vi "drawCircle.vi"(0 "reference":refnum<class "Graphics.lvclass">, 1 "rectangle":T1 {"height" format="%.2f"; "width" format="%.2f"; "y" format="%.2f"; "x" format="%.2f"}, 2 "lineWidth(1)":dbl=1.0 format="%.2f", 3 "color(if not used=default color)":u32=33554432 format="%.0x", 4 "fill?(F)":bool, 5 "error in (no error)":errorcluster) -> (14 "reference out":refnum<class "Graphics.lvclass">, 19 "error out":errorcluster)   [LabVIEW 2020, in "Graphics.lvclass"]
uses:
  <resource>/Framework/Providers/Open_GDS/UML/Graphics_class/Graphics.lvclass
  <resource>/Framework/Providers/Open_GDS/UML/General/Rectangle/Rectangle Rectangle2D.ctl
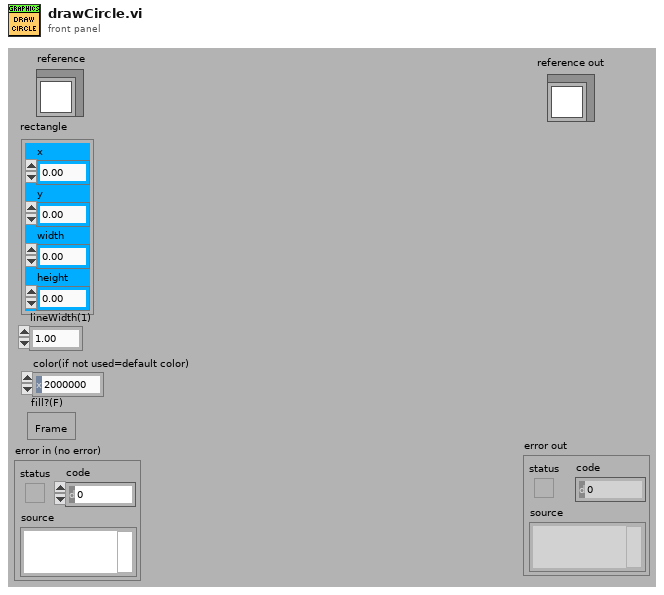
[diagram p1: front panel]
types:
  T1 = typedef "Rectangle Rectangle2D.ctl" = cluster{"x":dbl, "y":dbl, "width":dbl, "height":dbl}
  T2 = typedef "Graphics.lvclass/ObjectAttributes.ctl" = cluster{"drawColor":u32, "backgroundColor":u32, "font":T3, "fontType":T4, "picture":picture, "stroke":T5, "scaleX":dbl, "scaleY":dbl, "screenRef":refnum<vi>, "offsetX":dbl, "offsetY":dbl}
  T3 = typedef "Graphics.lvclass/FontType.ctl" = cluster{"Font Name:":string, "Size":i16, "Strikeout?":bool, "Italic?":bool, "Underline?":bool, "Outline?":bool, "Shadow?":bool, "Bold?":bool}
  T4 = typedef "Graphics.lvclass/LvFontType.ctl" = enum16{"User-specified Font", "Application Font", "System Font", "Dialog Font"}
  T5 = typedef "Graphics.lvclass/StrokeType.ctl" = enum16{"USE_DEFAULT", "SOLID", "DOTTED"}
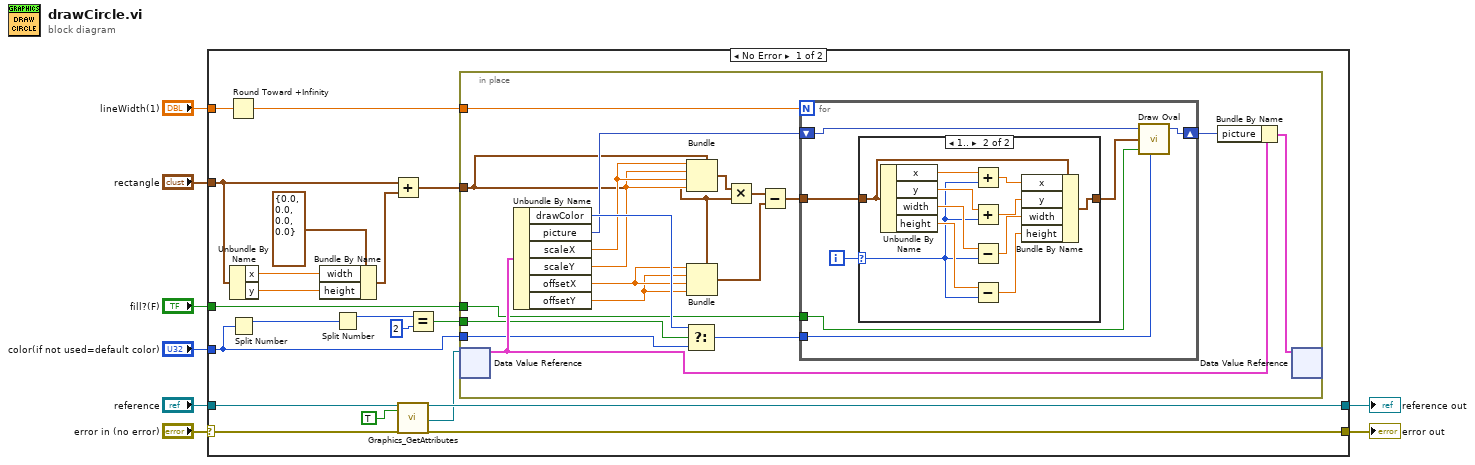
[diagram p0: block diagram]
diagram:
  n1 = case shown="No Error" "error in (no error)" {
    selector: "error in (no error)" -> [w25 w67]
    tunnel: "reference" -> [w28 w68]
    tunnel: [w27 w67] -> w7
    tunnel: [w26 w68] -> w6
    tunnel: "rectangle" -> [w24 _]
    tunnel: "lineWidth(1)" -> [w23 _]
    tunnel: "color(if not used=default color)" -> [w11 _]
    tunnel: "fill?(F)" -> [w12 _]
    frame No Error {
      n2 = Round Toward +Infinity(x=w23) -> (ceil(x): smallest int >= x=w13:dbl)
      n3 = Split Number(x=w11) -> (hi(x)=w22:u16)  [unwired: 1 out]
      n4 = Unbundle By Name(w24) -> ("x"=w18:dbl, "y"=w17:dbl)
      n5 = Bundle By Name(cluster=T1 {"x"=0.0, "y"=0.0, "width"=0.0, "height"=0.0} ("x"), "width"=w18, "height"=w17) -> (w16:T1)
      n6 = Split Number(x=w22) -> (hi(x)=w21:u8)  [unwired: 1 out]
      n7 = Add(x=w24, y=w16) -> (x+y=w9:T1)
      n8 = call <resource>:"Graphics_GetAttributes.vi"("reference in"=w28, "OnlyGetDvrReference(False)"=TRUE, "error in (no error)"=w25) -> ("reference out"=w26:refnum<class "Graphics.lvclass">, "DataRef"=w14:refnum<data-value>, "error out"=w27:errorcluster)  [unwired: 13 in, 1 out]
      n9 = Equal?(x=w21, y=u8 2) -> (x = y?=w10:bool)
      n10 = in-place {
        in-place-border: w13 -> [w38]
        in-place-border: w12 -> [w35]
        in-place-border: w11 -> [w34]
        in-place-border: w10 -> [w33]
        in-place-border: w9 -> [w29]
        n11 = in-place-dvr #1(w14) -> (w47:T2)  [unwired: 1 out]
        n12 = Unbundle By Name(w47) -> ("drawColor"=w44:u32, "picture"=w43:picture, "scaleX"=w42:dbl, "scaleY"=w41:dbl, "offsetX"=w40:dbl, "offsetY"=w39:dbl)
        n13 = Select(t=w44, s=w33, f=w34) -> (s? t:f=w36:u32)
        n14 = Bundle(cluster=w29, "x"=w42, "y"=w41, "width"=w42, "height"=w41) -> (w32:T1)
        n15 = Bundle(cluster=w29, "x"=w40, "y"=w39, "width"=w40, "height"=w39) -> (w31:T1)
        n16 = Multiply(x=w32, y=w29) -> (x*y=w30:T1)
        n17 = Subtract(x=w30, y=w31) -> (x-y=w37:T1)
        n18 = for {
          N: w38 -> [_]
          tunnel: w37 -> [w50]
          tunnel: w36 -> [w53]
          shift-right: [w52] -> w46
          shift-left: w43 -> [w54]
          tunnel: w35 -> [w48]
          i -> [w49]
          n19 = case shown="1.." w49 {
            selector: w49 -> [_ w56]
            tunnel: [w55 w58] -> w51
            tunnel: w50 -> [w55 w57]
            frame 0, Default {
            }
            frame 1.. {
              n20 = Unbundle By Name(w57) -> ("x"=w66:dbl, "y"=w65:dbl, "width"=w64:dbl, "height"=w63:dbl)
              n21 = Add(x=w66, y=w56) -> (x+y=w62:dbl)
              n22 = Add(x=w65, y=w56) -> (x+y=w61:dbl)
              n23 = Subtract(x=w64, y=w56) -> (x-y=w60:dbl)
              n24 = Subtract(x=w63, y=w56) -> (x-y=w59:dbl)
              n25 = Bundle By Name(cluster=w57, "x"=w62, "y"=w61, "width"=w60, "height"=w59) -> (w58:T1)
            }
          }
          n26 = call <vilib>:"Draw Oval.vi"("picture"=w54, "rect"=w51, "fill?(F)"=w48, "color(black)"=w53) -> ("new picture"=w52:picture)  [unwired: 1 in, 4 out]
        }
        n27 = Bundle By Name(cluster=w47, "picture"=w46) -> (w45:T2)
        n28 = in-place-dvr #1(w45) -> ()  [unwired: 2 out]
      }
    }
    frame Error {
    }
  }
  "reference out" <- w6
  "error out" <- w7
